vi "P0_AppVersion.vi"(11 "Inputs":string[](array[string])) -> (2 "Output/Failure":string, 3 "CLI Process Return Code":i32)   [LabVIEW 2026]
doc: "Slice 1.1 probe: reads Application Version Number of the running LabVIEW."
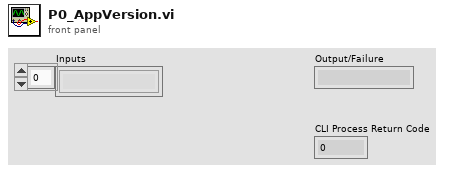
[diagram p1: front panel]
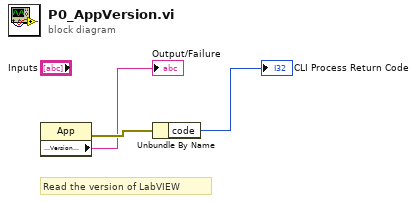
[diagram p0: block diagram]
diagram:
  # "Read the version of LabVIEW"
  n1 = property class="App"() -> (error out=w2:errorcluster, "Application:Version Number"=→"Output/Failure":string)  [unwired: 2 in, 1 out]
  n2 = Unbundle By Name(w2) -> ("code"=→"CLI Process Return Code":i32)
